vi "UDP Connection.vi"() -> ()   [LabVIEW 2026]
panel:
  in  "Numeric":i32
  in  "Blank Button":bool
  in  "String 2":string
  in  "String":string
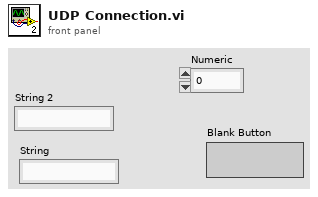
[diagram p1: front panel]
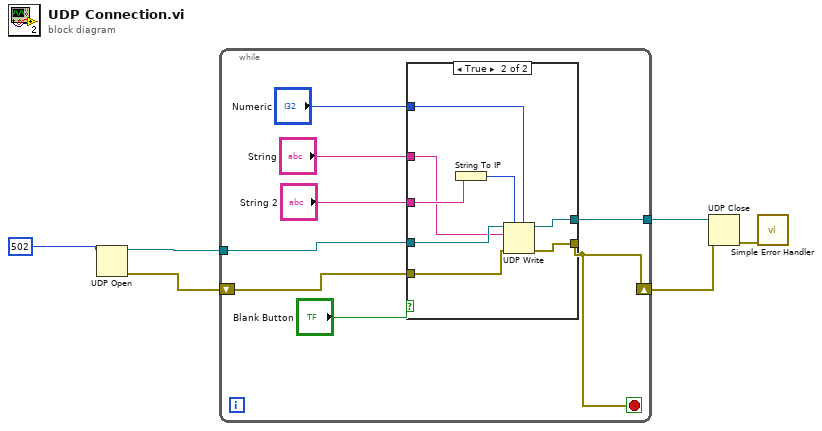
[diagram p0: block diagram]
diagram:
  n1 = UDP Open(11:502) -> (port=w5:refnum<k16>, 0:w2:errorcluster)  [unwired: 4 in, 1 out]
  n2 = while {
    tunnel: w5 -> [w13]
    tunnel: [w12] -> w4
    shift-right: [w7] -> w1
    shift-left: w2 -> [w8]
    stop <- w7 stop-if-true
    n3 = case shown="True" "Blank Button" {
      tunnel: [w15 w24] -> w7
      tunnel: w13 -> [w16 w23]
      tunnel: [w16 w22] -> w12
      tunnel: "String 2" -> [_ w20]
      tunnel: "String" -> [_ w19]
      tunnel: "Numeric" -> [_ w18]
      tunnel: w8 -> [w15 w17]
      frame False {
      }
      frame True {
        n4 = String To IP(1:w20) -> (0:w21:u32)
        n5 = UDP Write(address=w21, port or service name=w18, connection ID=w23, data in=w19, 8:w17) -> (error out=w24:errorcluster, 3:w22:refnum<k16>)  [unwired: 1 in]
      }
    }
  }
  n6 = UDP Close(connection ID=w4, 8:w1) -> (error out=w3:errorcluster)  [unwired: 1 out]
  n7 = call <vilib>:"Simple Error Handler.vi"("error in (no error)"=w3) -> ()  [unwired: 4 in, 5 out]
